vi "Build_Asylum_SetOutWave.vi"(6 "interpolation":i32, 8 "error in (no error)":errorcluster, 9 "Wave":cluster{"channelString":string, "wave":string}, 10 "eventString":string, 11 "whichBank":i32) -> (0 "error out":errorcluster, 3 "Command":string)   [LabVIEW 2019]
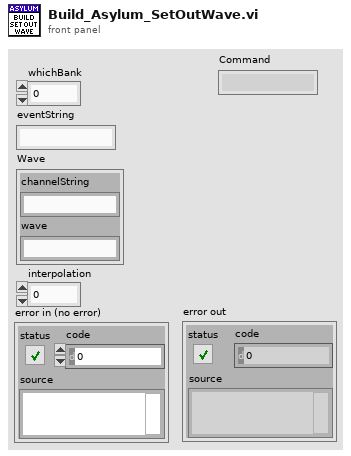
[diagram p1: front panel]
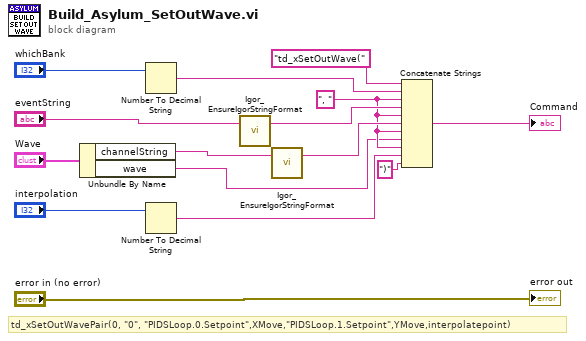
[diagram p0: block diagram]
diagram:
  w6 = ", " ("string")
  # "td_xSetOutWavePair(0, \"0\", \"PIDSLoop.0.Setpoint\",XMove,\"PIDSLoop.1.Setpoint\",YMove,interpolatepoint)"
  n1 = Unbundle By Name("Wave") -> ("channelString"=w11:string, "wave"=w2:string)
  n2 = Number To Decimal String(number="whichBank") -> (decimal integer string=w9:string)  [unwired: 1 in]
  n3 = Number To Decimal String(number="interpolation") -> (decimal integer string=w5:string)  [unwired: 1 in]
  n4 = call <userlib>:"Igor_EnsureIgorStringFormat.vi"("Value"="eventString") -> ("Value"=w8:string)  [unwired: 2 in]
  n5 = call <userlib>:"Igor_EnsureIgorStringFormat.vi"("Value"=w11) -> ("Value"=w7:string)  [unwired: 2 in]
  n6 = Concatenate Strings("td_xSetOutWave(" ("string"), w9, w6, w8, w6, w7, w6, w2, w6, w5, ")" ("string")) -> (→"Command":string)
  "error out" <- "error in (no error)"
